vi "GetSetGainAuto.vi"(7 "Set?":bool, 8 "error in (no error)":errorcluster, 10 "Auto Mode":T1, 11 "Camera in":refnum<class "Camera.lvclass">) -> (0 "error out":errorcluster, 2 "Mode":T1)   [LabVIEW 2020, in "Camera.lvclass"]
uses:
  Camera.lvclass
  Auto Mode.ctl
  Camera.lvclass/Camera.ctl
  bin/gindustrialcam_32-1.dll
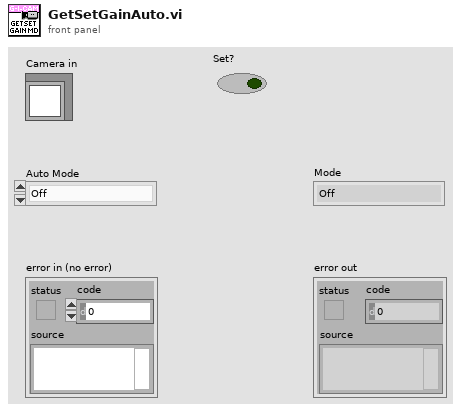
[diagram p1: front panel]
types:
  T1 = typedef "Camera.lvclass/Auto Mode.ctl" = enum8{"Off", "Once", "Continuous"}
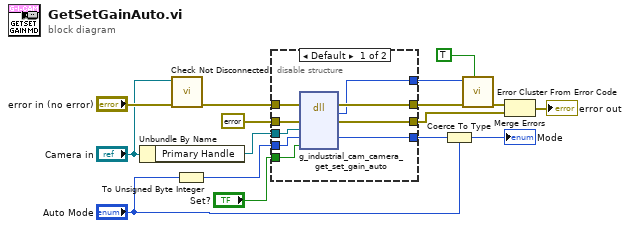
[diagram p0: block diagram]
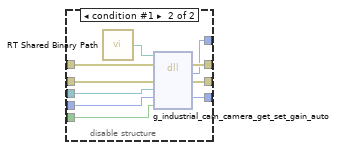
[diagram p2: hidden frame]
diagram:
  n1 = Unbundle By Name("Camera in") -> ("Primary Handle"=w7:refnum<data-value>)
  n2 = call "Check Not Disconnected.vi"("error in (no error)"="error in (no error)", "Camera in"="Camera in") -> ("error out"=w2:errorcluster)  [unwired: 9 in]
  n3 = To Unsigned Byte Integer(number="Auto Mode") -> (unsigned 8bit integer=w6:u8)
  n4 = disable-structure shown="Default" {
    disable-tunnel: [w25 w35] -> w16
    disable-tunnel: [w24 w34] -> w15
    disable-tunnel: [w23 w33] -> w13
    disable-tunnel: errorcluster {"status"=FALSE, "code"=0, "source"=""} ("error constant") -> [w22 w32]
    disable-tunnel: "Set?" -> [w21 w31]
    disable-tunnel: w7 -> [w20 w30]
    disable-tunnel: w6 -> [w19 w29]
    disable-tunnel: [w18 w28] -> w5
    disable-tunnel: w2 -> [w17 w27]
    frame condition #0 (active) {
      n5 = dll-call lib="C:/serenial/lib/g-industrial-camera/LabVIEW/g_industrial_cam/bin/gindustrialcam_*-1.*" fn="g_industrial_cam_camera_get_set_gain_auto"(error in=w17, "err"=w22, "edvr"=w20, "value"=w19, "set"=w21) -> (error out=w25:errorcluster, "Mg_Error"=w24:i32, "err"=w23:errorcluster, "value"=w18:u8)  [unwired: 4 in, 1 out]
    }
    frame condition #1 {
      n6 = call "RT Shared Binary Path.vi"() -> ("Path"=w26:path)
      n7 = dll-call lib="C:/serenial/lib/g-industrial-camera/LabVIEW/g_industrial_cam/bin/gindustrialcam_*-1.*" fn="g_industrial_cam_camera_get_set_gain_auto"(path in=w26, error in=w27, "err"=w32, "edvr"=w30, "value"=w29, "set"=w31) -> (error out=w35:errorcluster, "Mg_Error"=w34:i32, "err"=w33:errorcluster, "value"=w28:u8)  [unwired: 3 in, 1 out]
    }
  }
  n8 = Coerce To Type(0:w5, 1:"Auto Mode") -> (2:→"Mode":T1)
  n9 = call <vilib>:"Error Cluster From Error Code.vi"("show call chain? (False)"=TRUE, "error in (no error)"=w16, "error code (0)"=w15) -> ("error out"=w14:errorcluster)  [unwired: 6 in]
  n10 = Merge Errors(w14, w13) -> (→"error out":errorcluster)
